vi "Dispose.vi"(8 "error in (no error)":errorcluster, 11 "WebView2 Control in":refnum<class "WebView2 Control.lvclass">) -> (0 "error out":errorcluster)   [LabVIEW 2020, in "WebView2.lvlib" / "WebView2 Control.lvclass"]
uses:
  WebView2 Control.lvclass
  WebView2 Control.lvclass/WebView2 Control.ctl
  E:/Labview/LV 2023/PPL/PPL Builder/Libs/LV-WebView2/Source/Libs/Microsoft.Web.WebView2.Core.dll
  Libs/Microsoft.Web.WebView2.Core.dll
  WebView2 Event Filter Interface/WebView2 Event Filter Interface.lvclass
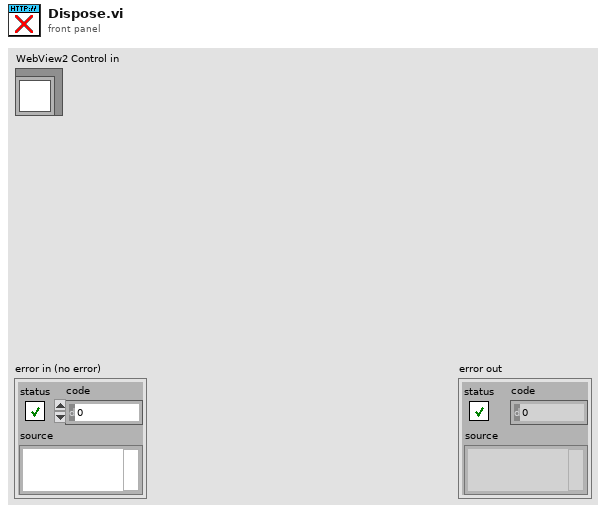
[diagram p1: front panel]
types:
  T1 = typedef "WebView2.lvlib/WebView2 Control.lvclass/Events.ctl" = cluster{"Navigation Complete Event":refnum<user-event>, "Source Changed Event":refnum<user-event>, "Document Title Changed Event":refnum<user-event>, "Status Bar Text Changed":refnum<user-event>, "Web Message Received":refnum<user-event>, "Window Close Requested":refnum<user-event>, "DOM Loaded":refnum<user-event>, "Navigation Started Event":refnum<user-event>, "New Window Requested Event":refnum<user-event>, "Content Loading Event":refnum<user-event>}
  T2 = typedef "WebView2.lvlib/WebView2 Control.lvclass/Res.ctl" = cluster{"WebView2":refnum<k24>, "Webview2 Core":refnum<k24>, "event callback":refnum<k27>, "Environment":refnum<k24>}
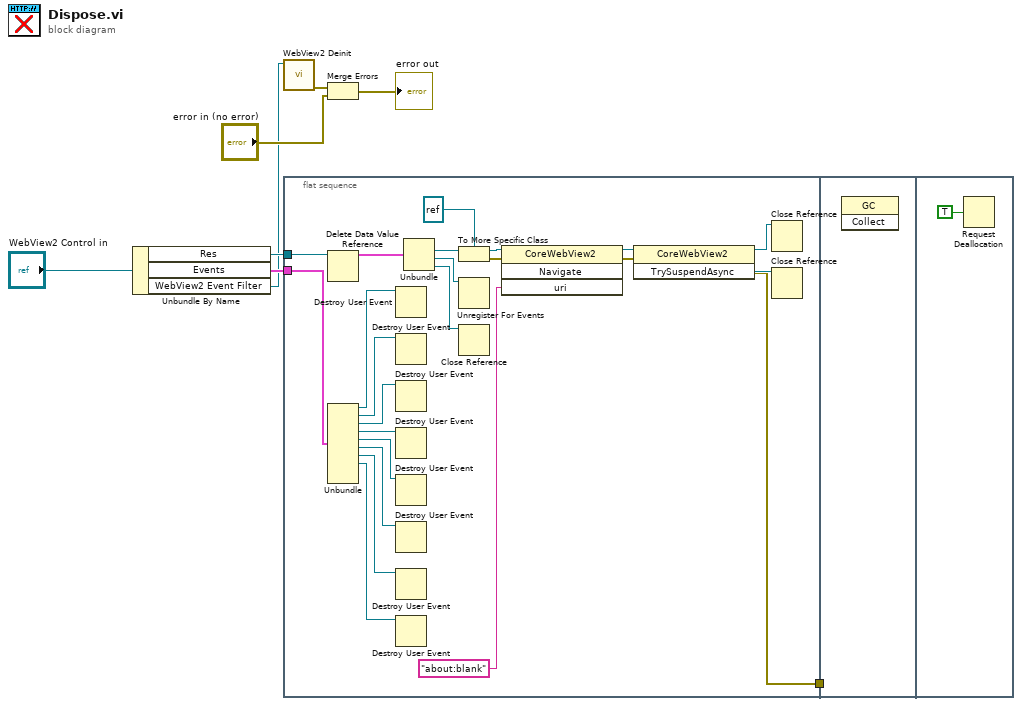
[diagram p0: block diagram]
diagram:
  n1 = Unbundle By Name("WebView2 Control in") -> ("Res"=w6:refnum<data-value>, "Events"=w5:T1, "WebView2 Event Filter"=w3:refnum<class "WebView2 Event Filter Interface.lvclass">)
  n2 = call-dynamic "WebView2 Deinit.vi"("WebView2 Event Filter Interface in"=w3) -> ("error out"=w1:errorcluster)  [unwired: 10 in]
  n3 = flat-sequence {
    tunnel: w6 -> [w13]
    tunnel: w5 -> [w31]
    tunnel: [w9] -> w4
    tunnel: w4 -> [_]
    frame #0 {
      n4 = Delete Data Value Reference(data value reference=w13) -> (data value=w14:T2)  [unwired: 1 in, 1 out]
      n5 = Unbundle(w31) -> ("Navigation Complete Event"=w30:refnum<user-event>, "Source Changed Event"=w29:refnum<user-event>, "Document Title Changed Event"=w28:refnum<user-event>, "Status Bar Text Changed"=w27:refnum<user-event>, "Web Message Received"=w26:refnum<user-event>, "Window Close Requested"=w25:refnum<user-event>, "DOM Loaded"=w24:refnum<user-event>, "Navigation Started Event"=w23:refnum<user-event>)  [unwired: 2 out]
      n6 = Destroy User Event(user event=w30) -> ()  [unwired: 1 in, 1 out]
      n7 = Destroy User Event(user event=w29) -> ()  [unwired: 1 in, 1 out]
      n8 = Destroy User Event(user event=w28) -> ()  [unwired: 1 in, 1 out]
      n9 = Destroy User Event(user event=w27) -> ()  [unwired: 1 in, 1 out]
      n10 = Destroy User Event(user event=w26) -> ()  [unwired: 1 in, 1 out]
      n11 = Destroy User Event(user event=w25) -> ()  [unwired: 1 in, 1 out]
      n12 = Destroy User Event(user event=w24) -> ()  [unwired: 1 in, 1 out]
      n13 = Destroy User Event(user event=w23) -> ()  [unwired: 1 in, 1 out]
      n14 = Unbundle(w14) -> ("Webview2 Core"=w16:refnum<k24>, "event callback"=w22:refnum<k27>, "Environment"=w21:refnum<k24>)  [unwired: 1 out]
      n15 = To More Specific Class(target class=refnum<k24> refnum ("Webview2 Core"), reference=w16) -> (specific class reference=w12:refnum<k24>, error out=w10:errorcluster)  [unwired: 1 in]
      n16 = Unregister For Events(event registration refnum=w22) -> ()  [unwired: 1 in, 1 out]
      n17 = Close Reference(reference=w21) -> ()  [unwired: 1 in, 1 out]
      n18 = invoke class="CoreWebView2" method="Navigate"(reference=w12, error in=w10, "uri"="about:blank") -> (reference out=w19:refnum<k24>, error out=w20:errorcluster)  [unwired: 1 in, 2 out]
      n19 = invoke class="CoreWebView2" method="TrySuspendAsync"(reference=w19, error in=w20) -> (reference out=w17:refnum<k24>, error out=w9:errorcluster, "TrySuspendAsync"=w18:refnum<k24>)  [unwired: 1 in]
      n20 = Close Reference(reference=w17) -> ()  [unwired: 1 in, 1 out]
      n21 = Close Reference(reference=w18) -> ()  [unwired: 1 in, 1 out]
    }
    frame #1 {
      n22 = invoke class="GC" method="Collect"() -> ()  [unwired: 3 in, 3 out]
    }
    frame #2 {
      n23 = Request Deallocation(TRUE ("flag")) -> ()
    }
  }
  n24 = Merge Errors(w1, "error in (no error)") -> (→"error out":errorcluster)
